vi "NanonisGetScanPixels.vi"(8 "error in (no error)":errorcluster, 11 "String input":string="string test") -> (0 "error out":errorcluster, 3 "String output":string)   [LabVIEW 2011]
uses:
  <userlib>/Nanonis Prog Interface/Nanonis Prog Interface.lvlib
panel:
  out "Application ref out":refnum<vi>
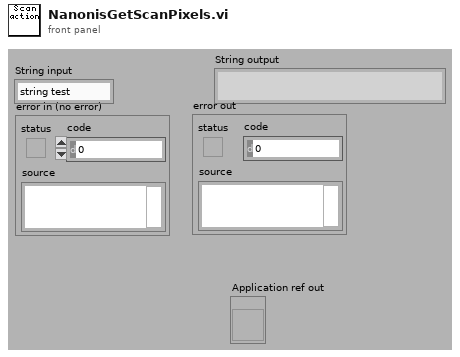
[diagram p1: front panel]
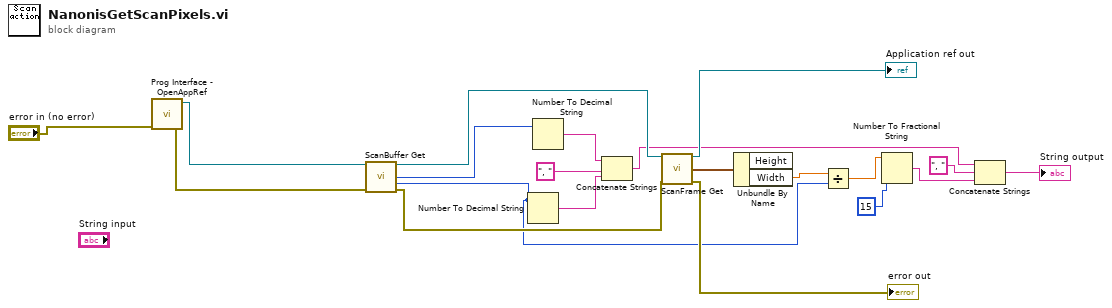
[diagram p0: block diagram]
diagram:
  n1 = call <userlib>:"Prog Interface - OpenAppRef.vi"("Error in (no error)"="error in (no error)") -> ("Error out"=w18:errorcluster, "Application reference"=w19:refnum<vi>)  [unwired: 5 in]
  n2 = call <userlib>:"ScanBuffer Get.vi"("Application ref in"=w19, "error in (no error)"=w18) -> ("Application ref out"=w12:refnum<vi>, "Pixels/line"=w17:i32, "Lines"=w7:i32, "error out"=w13:errorcluster)  [unwired: 9 in, 1 out]
  n3 = Number To Decimal String(number=w7) -> (decimal integer string=w14:string)  [unwired: 1 in]
  n4 = Number To Decimal String(number=w17) -> (decimal integer string=w15:string)  [unwired: 1 in]
  n5 = Concatenate Strings(w15, ", ", w14) -> (w3:string)
  n6 = call <userlib>:"ScanFrame Get.vi"("Application ref in"=w12, "error in (no error)"=w13) -> ("Application ref out"=→"Application ref out":refnum<vi>, "Size (m)"=w9:cluster{"Width":sgl, "Height":sgl}, "error out"=→"error out":errorcluster)  [unwired: 9 in, 2 out]
  n7 = Unbundle By Name(w9) -> ("Width"=w8:sgl)  [unwired: 1 out]
  n8 = Divide(x=w8, y=w7) -> (x/y=w6:sgl)
  n9 = Number To Fractional String(number=w6, precision (6)=15) -> (F-format string=w2:string)  [unwired: 2 in]
  n10 = Concatenate Strings(w3, ", ", w2) -> (→"String output":string)
